vi "Enqueue Blocks.vi"(10 "data":u8[](array[numeric]) format="%.0x", 11 "Blocks queue":refnum<queue>) -> ()   [LabVIEW 2013, in "MD5.lvlib" / "MD5.lvclass"]
uses:
  MD5.lvclass
  Data-vector.ctl
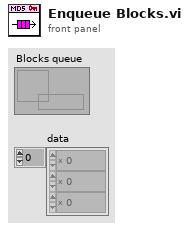
[diagram p1: front panel]
types:
  T1 = typedef "MD5.lvlib/MD5.lvclass/Data-vector.ctl" = cluster{"Data[ ]":u8[], "end":bool}
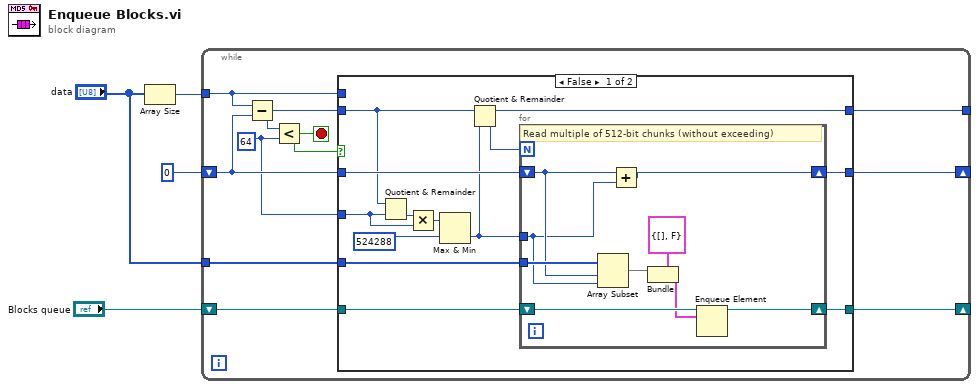
[diagram p0: block diagram]
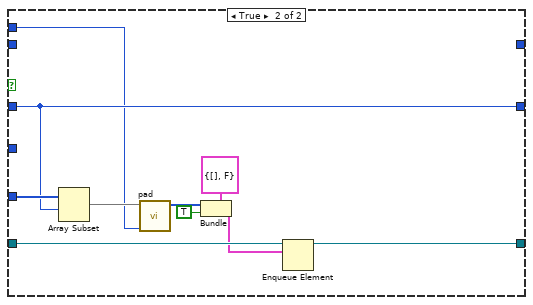
[diagram p2: hidden frame]
diagram:
  n1 = Array Size(array="data") -> (size(s)=w1:i32)
  n2 = while {
    shift-right: [w10] -> _
    shift-left: 0 ("offset") -> [w12]
    tunnel: w1 -> [w5]
    tunnel: [w11] -> _
    tunnel: "data" -> [w9]
    shift-right: [w13] -> _
    shift-left: "Blocks queue" -> [w14]
    stop <- w6 stop-if-true
    w7 = 64 ("y")
    n3 = Subtract(x=w5, y=w12) -> (x-y=w8:i32)
    n4 = Less?(x=w8, y=w7) -> (x < y?=w6:bool)
    n5 = case shown="False" w6 {
      tunnel: w14 -> [w27 w42]
      tunnel: [w26 w41] -> w13
      tunnel: w12 -> [w25 w45]
      tunnel: [w19 _] -> w11
      tunnel: [w18 w45] -> w10
      tunnel: w9 -> [w17 w46]
      tunnel: w8 -> [w16 _]
      tunnel: w7 -> [w15 _]
      tunnel: w5 -> [_ w43]
      frame False {
        n6 = Quotient & Remainder(x=w16, y=w15) -> (floor(x/y)=w24:i32)  [unwired: 1 out]
        n7 = Multiply(x=w24, y=w15) -> (x*y=w23:i32)
        n8 = Max & Min(x=w23, y=524288) -> (min(x,y)=w20:i32)  [unwired: 1 out]
        n9 = Quotient & Remainder(x=w16, y=w20) -> (x-y*floor(x/y)=w19:i32, floor(x/y)=w21:i32)
        n10 = for {
          N: w21 -> [_]
          shift-right: [w35] -> w26
          shift-left: w27 -> [w36]
          shift-right: [w28] -> w18
          shift-left: w25 -> [w30]
          tunnel: w20 -> [w29]
          tunnel: w17 -> [w32]
          # "Read multiple of 512-bit chunks (without exceeding)"
          n11 = Array Subset(array=w32, index=w30, length=w29) -> (w31:u8[])
          n12 = Add(x=w30, y=w29) -> (x+y=w28:i32)
          n13 = Bundle(cluster=T1 {"Data[ ]"=[], "end"=FALSE}, "Data[ ]"=w31) -> (w33:T1)  [unwired: 1 in]
          n14 = Enqueue Element(queue=w36, element=w33) -> (queue out=w35:refnum<queue>)  [unwired: 2 in, 2 out]
        }
      }
      frame True {
        n15 = Array Subset(array=w46, index=w45) -> (w44:u8[])  [unwired: 1 in]
        n16 = call "pad.vi"("data length"=w43, "Last Block"=w44) -> ("Padding"=w39:u8[])  [unwired: 8 in, 1 out]
        n17 = Bundle(cluster=T1 {"Data[ ]"=[], "end"=FALSE}, "Data[ ]"=w39, "end"=TRUE) -> (w37:T1)
        n18 = Enqueue Element(queue=w42, element=w37) -> (queue out=w41:refnum<queue>)  [unwired: 2 in, 2 out]
      }
    }
  }
